vi "Record Frame Mouse Metadata.vi"(0 "Module ID":i32=-1, 1 "button info":T2, 2 "Relative Time (User Event)":dbl, 5 "Sample Number":u32, 7 "Relative Time (Frame 0)":dbl, 9 "KeyboardAndMouseData.Keyboard Keys Pressed":T1[](array[typedef]), 11 "error in":errorcluster, 12 "axis info":T3, 13 "key mode":enum16{"RELATIVE", "ABSOLUTE"}(ring), 14 "KeyboardAndMouseData.Frame Number":u32) -> (15 "error out":errorcluster)   [LabVIEW 2026, in "UserEventRecorder.lvlib"]
doc: "_____\nCreated using DQMH Framework: Event Scripter 7.1.2.1547."
uses:
  UserEventRecorder.lvlib
  Record Frame Mouse Metadata Argument--cluster.ctl
  dependencies.lvlibp/dependencies/src/KeyboardAndMouseDataAcquisition.ctl
  dependencies.lvlibp
  dependencies.lvlibp/dependencies/src/KeyType.ctl
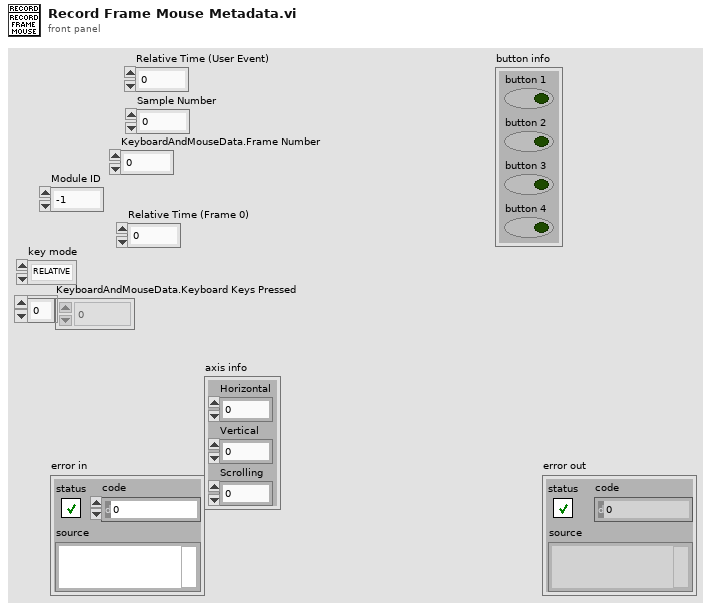
[diagram p1: front panel]
types:
  T1 = typedef "dependencies.lvlibp/KeyType.ctl" = enum16{"0", "1", "2", "3", "4", "5", "6", "7", "8", "9", "A", "B", "C", "D", "E", "F", "G", "H", "I", "J", "K", "L", "M", "N", "O", "P", "Q", "R", "S", "T", "U", "V", "W", "X", "Y", "Z", "F1", "F2", "F3", "F4", "F5", "F6", "F7", "F8", "F9", "F10", "F11", "F12", "F13", "F14", "F15", "ADD", "BACK", "BACKSLASH", "CAPITAL", "COMMA", "DECIMAL", "DELETE", "DIVIDE", "DOWN", "END", "EQUALS", "ESCAPE", "GRAVE (`)", "HOME", "INSERT", "LBRACKET", "LCONTROL", "LEFT", "L ALT", "LSHIFT", "LWIN", "MINUS", "MULTIPLY", "NEXT", "NUMLOCK", "NUMPAD_0", "NUMPAD_1", "NUMPAD_2", "NUMPAD_3", "NUMPAD_4", "NUMPAD_5", "NUMPAD_6", "NUMPAD_7", "NUMPAD_8", "NUMPAD_9", "PAUSE", "PERIOD", "PRIOR (PG UP)", "RBRACKET", "RCONTROL", "RETURN", "RIGHT", "R ALT", "RSHIFT", "RWIN", "SCROLL", "SEMICOLON", "SLASH", "SPACE", "SUBTRACT", "TAB", "UP", "ENTER (num pad)", "' (quote)"}
  T2 = cluster{"button 1":bool, "button 2":bool, "button 3":bool, "button 4":bool}
  T3 = cluster{"Horizontal":i32, "Vertical":i32, "Scrolling":i32}
  T4 = typedef "UserEventRecorder.lvlib/Record Frame Mouse Metadata Argument--cluster.ctl" = cluster{"Module ID":i32, "KeyboardAndMouseData":T5}
  T5 = typedef "dependencies.lvlibp/KeyboardAndMouseDataAcquisition.ctl" = cluster{"axis info":cluster{"Horizontal":i32, "Vertical":i32, "Scrolling":i32}, "button info":cluster{"button 1":bool, "button 2":bool, "button 3":bool, "button 4":bool}, "Relative Time (User Event)":dbl, "Sample Number":u32, "Relative Time (Frame 0)":dbl, "key mode":enum16{"RELATIVE", "ABSOLUTE"}, "Frame Number":u32, "Keyboard KeyPressed":enum16{"0", "1", "2", "3", "4", "5", "6", "7", "8", "9", "A", "B", "C", "D", "E", "F", "G", "H", "I", "J", "K", "L", "M", "N", "O", "P", "Q", "R", "S", "T", "U", "V", "W", "X", "Y", "Z", "F1", "F2", "F3", "F4", "F5", "F6", "F7", "F8", "F9", "F10", "F11", "F12", "F13", "F14", "F15", "ADD", "BACK", "BACKSLASH", "CAPITAL", "COMMA", "DECIMAL", "DELETE", "DIVIDE", "DOWN", "END", "EQUALS", "ESCAPE", "GRAVE (`)", "HOME", "INSERT", "LBRACKET", "LCONTROL", "LEFT", "L ALT", "LSHIFT", "LWIN", "MINUS", "MULTIPLY", "NEXT", "NUMLOCK", "NUMPAD_0", "NUMPAD_1", "NUMPAD_2", "NUMPAD_3", "NUMPAD_4", "NUMPAD_5", "NUMPAD_6", "NUMPAD_7", "NUMPAD_8", "NUMPAD_9", "PAUSE", "PERIOD", "PRIOR (PG UP)", "RBRACKET", "RCONTROL", "RETURN", "RIGHT", "R ALT", "RSHIFT", "RWIN", "SCROLL", "SEMICOLON", "SLASH", "SPACE", "SUBTRACT", "TAB", "UP", "ENTER (num pad)", "' (quote)"}, "Keyboard No Op":bool}
  T6 = typedef "UserEventRecorder.lvlib/Request Events--cluster.ctl" = cluster{"Stop Module":refnum<user-event>, "Show Panel":refnum<user-event>, "Hide Panel":refnum<user-event>, "Show Diagram":refnum<user-event>, "Get Module Execution Status":refnum<user-event>, "Record Frame Mouse Metadata":refnum<user-event>, "Local Instance":T7}
  T7 = typedef "UserEventRecorder.lvlib/Local Instance Request Events--cluster.ctl" = cluster{"Test Event Triggered":refnum<user-event>}
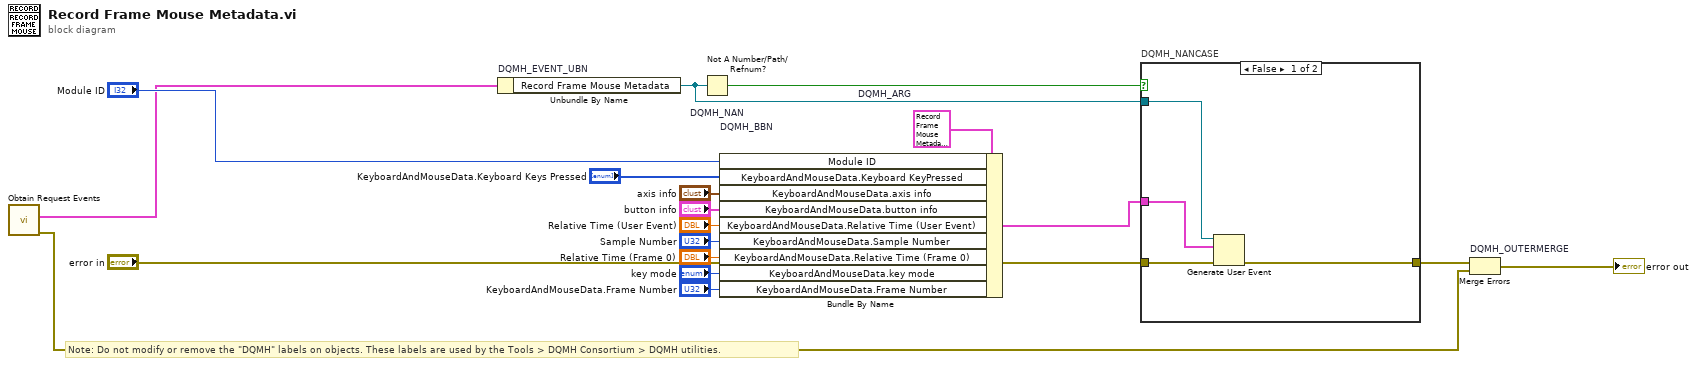
[diagram p0: block diagram]
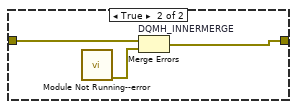
[diagram p2: hidden frame]
diagram:
  w13 = T4 {"Module ID"=-1, "KeyboardAndMouseData"={"axis info"={"Horizontal"=0, "Vertical"=0, "Scrolling"=0}, "button info"={"button 1"=FALSE, "button 2"=FALSE, "button 3"=FALSE, "button 4"=FALSE}, "Relative Time (User Event)"=0.0, "Sample Number"=0, "Relative Time (Frame 0)"=0.0, "key mode"=enum."ABSOLUTE", "Frame Number"=0, "Keyboard KeyPressed"=enum."RIGHT", "Keyboard No Op"=FALSE}}  # DQMH_ARG
  # "Note: Do not modify or remove the \"DQMH\" labels on objects. These labels are used by the Tools > DQMH Consortium > DQMH utilities."
  n1 = call "Obtain Request Events.vi"() -> ("error out"=w11:errorcluster, "UserEventRecorder Request Events"=w10:T6)  [unwired: 10 in]
  n2 = Unbundle By Name "DQMH_EVENT_UBN"(w10) -> ("Record Frame Mouse Metadata"=w15:refnum<user-event>)
  n3 = Not A Number/Path/Refnum? "DQMH_NAN"(number/path/refnum=w15) -> (NaN/Path/Refnum?=w16:bool)
  n4 = Bundle By Name "DQMH_BBN"(cluster=w13, "Module ID"="Module ID", "KeyboardAndMouseData.Keyboard KeyPressed"="KeyboardAndMouseData.Keyboard Keys Pressed", "KeyboardAndMouseData.axis info"="axis info", "KeyboardAndMouseData.button info"="button info", "KeyboardAndMouseData.Relative Time (User Event)"="Relative Time (User Event)", "KeyboardAndMouseData.Sample Number"="Sample Number", "KeyboardAndMouseData.Relative Time (Frame 0)"="Relative Time (Frame 0)", "KeyboardAndMouseData.key mode"="key mode", "KeyboardAndMouseData.Frame Number"="KeyboardAndMouseData.Frame Number") -> (w17:T4)
  n5 = case "DQMH_NANCASE" shown="False" w16 {
    tunnel: "error in" -> [w22 w25]
    tunnel: [w21 w24] -> w14
    tunnel: w15 -> [w20 _]
    tunnel: w17 -> [w19 _]
    frame False {
      n6 = Generate User Event(user event=w20, event data cluster=w19, error in=w22) -> (error out=w21:errorcluster)  [unwired: 1 in, 1 out]
    }
    frame True {
      n7 = call "Module Not Running--error.vi"() -> ("error out"=w23:errorcluster)  [unwired: 11 in]
      n8 = Merge Errors "DQMH_INNERMERGE"(w25, w23) -> (w24:errorcluster)
    }
  }
  n9 = Merge Errors "DQMH_OUTERMERGE"(w14, w11) -> (→"error out":errorcluster)
